vi "UNO Q PinMode.vi"(8 "error in (no error)":errorcluster, 9 "OUTPUT":bool, 10 "Digital pin":T1, 11 "UNO Q Session in":T2={"HTTP client"=refnum, "Base URL"="", "Connected"=TRUE}) -> (0 "error out":errorcluster, 3 "UNO Q Session out":T2={"HTTP client"=refnum, "Base URL"="", "Connected"=TRUE}, 4 "status":i32, 6 "error":string)   [LabVIEW 2021]
uses:
  UNO Q Session.ctl
  <vilib>/httpClient/ClientHandle.ctl
  Dpin typedef.ctl
  ERR typedef.ctl
  <vilib>/httpClient/POSTBuffer.vi
  <vilib>/httpClient/LabVIEWHTTPClient.lvlib
panel:
  out "headers":string
  out "body":string
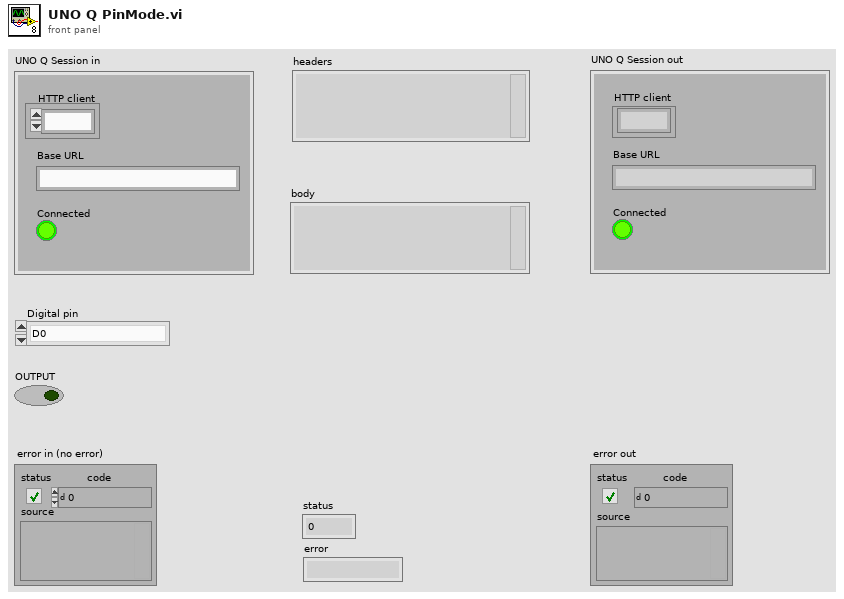
[diagram p1: front panel]
types:
  T1 = typedef "Dpin typedef.ctl" = enum16{"D0", "D1", "D2", "D3", "D4", "D5", "D6", "D7", "D8", "D9", "D10", "D11", "D12", "D13"}
  T2 = typedef "UNO Q Session.ctl" = cluster{"HTTP client":T3, "Base URL":string, "Connected":bool}
  T3 = typedef "LabVIEWHTTPClient.lvlib/ClientHandle.ctl" = refnum<k1>
  T4 = typedef "ERR typedef.ctl" = enum16{"STATUS OK", "STATUS INVALID ARGUMENT", "STATUS NOT IMPLEMENTED", "STATUS RUNTIME ERROR"}
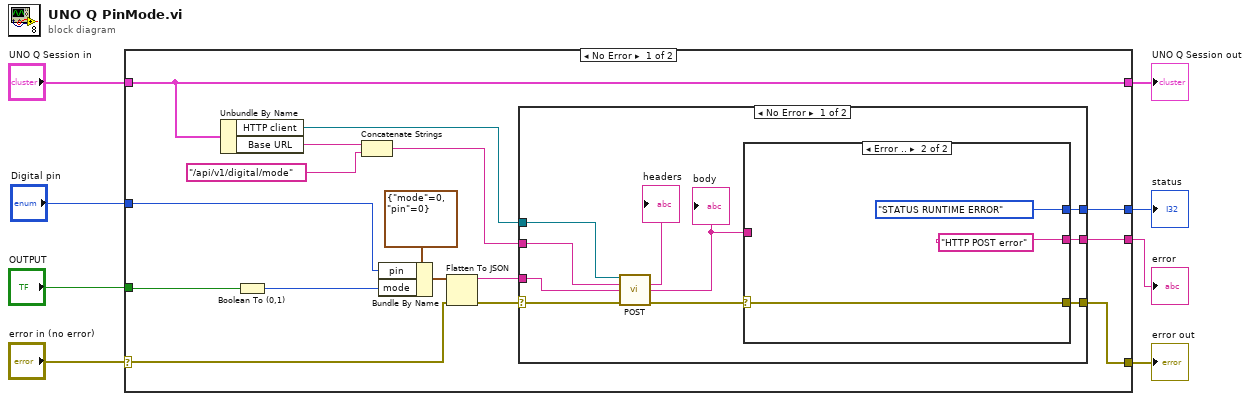
[diagram p0: block diagram]
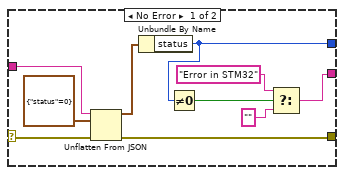
[diagram p2: hidden frame]
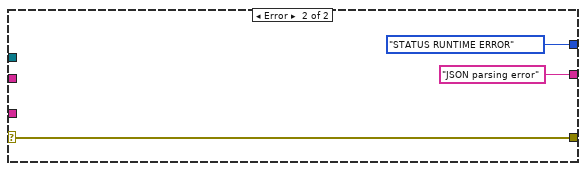
[diagram p3: hidden frame]
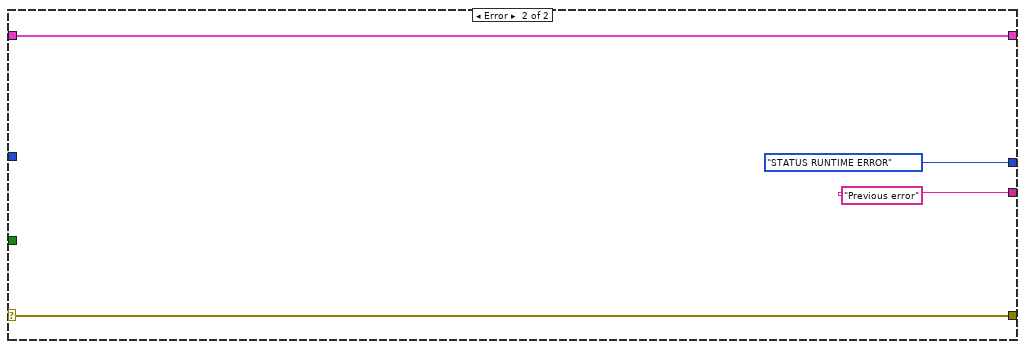
[diagram p4: hidden frame]
diagram:
  n1 = case shown="No Error" "error in (no error)" {
    selector: "error in (no error)" -> [w17 w54]
    tunnel: [w15 w54] -> w7
    tunnel: "UNO Q Session in" -> [w21 w53]
    tunnel: [w21 w53] -> w5
    tunnel: "OUTPUT" -> [w10 _]
    tunnel: [w14 ERR_typedef."STATUS RUNTIME ERROR" ("Error code")] -> w3
    tunnel: [w13 "Previous error" ("error")] -> w2
    tunnel: "Digital pin" -> [w11 _]
    frame No Error {
      n2 = Unbundle By Name(w21) -> ("HTTP client"=w20:T3, "Base URL"=w23:string)
      n3 = Boolean To (0,1)(Boolean=w10) -> (0, 1=w9:i16)
      n4 = Concatenate Strings(w23, "/api/v1/digital/mode" ("string")) -> (w19:string)
      n5 = Bundle By Name(cluster=cluster{"mode":i32, "pin":i32} {"mode"=0, "pin"=0}, "pin"=w11, "mode"=w9) -> (w24:cluster{"mode":i32, "pin":i32})
      n6 = Flatten To JSON(anything=w24, error in (no error)=w17) -> (JSON string=w18:string, 11:w16:errorcluster)  [unwired: 1 in]
      n7 = case shown="No Error" w16 {
        selector: w16 -> [w30 w50]
        tunnel: w20 -> [w34 _]
        tunnel: w19 -> [w33 _]
        tunnel: w18 -> [w32 _]
        tunnel: [w27 w50] -> w15
        tunnel: [w26 ERR_typedef."STATUS RUNTIME ERROR" ("Error code")] -> w14
        tunnel: [w25 "JSON parsing error" ("error")] -> w13
        frame No Error {
          n8 = call-poly <vilib>:"POST.vi"("client handle"=w34, "url"=w33, "buffer"=w32, "error in (no error)"=w30) -> ("headers"=→"headers":string, "body"=w28:string, "error out"=w29:errorcluster)  [unwired: 8 in, 1 out]
          "body" <- w28
          n9 = case shown="Error .." w29 {
            selector: w29 -> [w44 w47]
            tunnel: w28 -> [w43 _]
            tunnel: [w42 w47] -> w27
            tunnel: [w40 ERR_typedef."STATUS RUNTIME ERROR" ("Error code")] -> w26
            tunnel: [w36 "HTTP POST error" ("error")] -> w25
            frame No Error {
              n10 = Unflatten From JSON(JSON string=w43, type and defaults=cluster{"status":i32} {"status"=0}, error in (no error)=w44) -> (value=w39:cluster{"status":i32}, error out=w42:errorcluster)  [unwired: 4 in]
              n11 = Unbundle By Name(w39) -> ("status"=w40:i32)
              n12 = Not Equal To 0?(x=w40) -> (x != 0?=w38:bool)
              n13 = Select(t="Error in STM32", s=w38, f="") -> (s? t:f=w36:string)
            }
            frame Error {
            }
          }
        }
        frame Error {
        }
      }
    }
    frame Error {
    }
  }
  "error out" <- w7
  "UNO Q Session out" <- w5
  "status" <- w3
  "error" <- w2
